vi "Send TDF File List Response.vi"(8 "error in (no error)":errorcluster caption="에러 입력(에러 없음)", 9 "TDF File List":string[](array[string]), 10 "id":string, 11 "Instrument Manager 입력":refnum<class "Instrument Manager.lvclass">) -> (0 "error out":errorcluster caption="에러 출력", 3 "Instrument Manager 출력":refnum<class "Instrument Manager.lvclass">)   [LabVIEW 2023, in "Instrument Manager.lvclass"]
uses:
  Instrument Manager.lvclass
  TDF File List Response.ctl
  Instrument Manager.lvclass/Instrument Manager.ctl
  Error Response.ctl
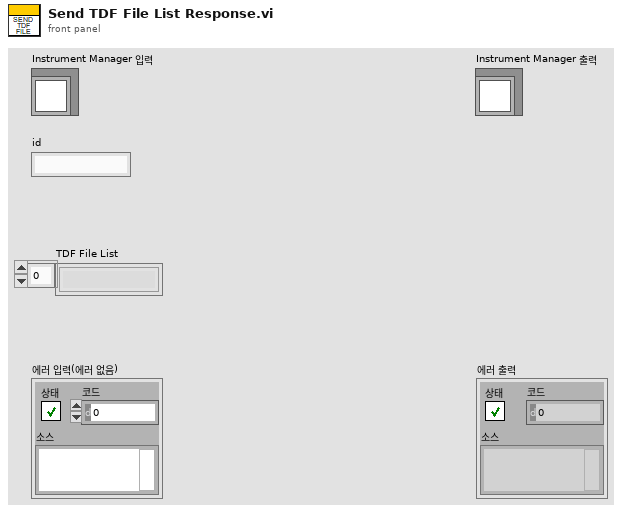
[diagram p1: front panel]
types:
  T1 = typedef "Instrument Manager.lvclass/TDF File List Response.ctl" = cluster{"type":string, "id":string, "status":string, "Result":cluster{"TDF File List":string[]}}
  T2 = cluster{"Reader Q":refnum<queue>, "Writer Q":refnum<queue>}
  T3 = typedef "Instrument Manager.lvclass/Error Response.ctl" = cluster{"type":string, "id":string, "status":string, "error out":errorcluster}
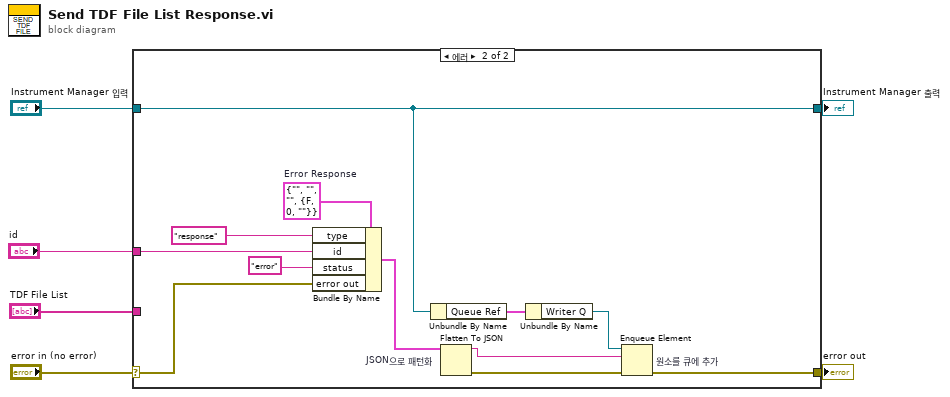
[diagram p0: block diagram]
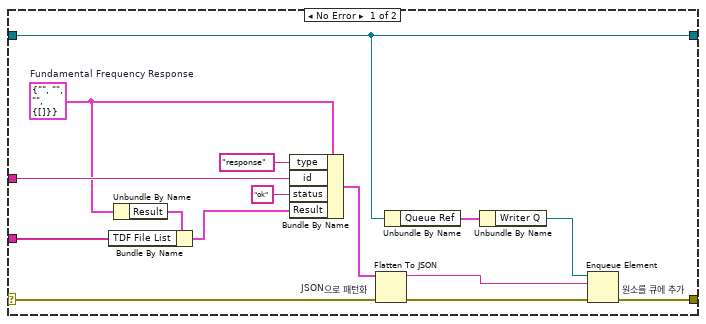
[diagram p2: hidden frame]
diagram:
  n1 = case shown="에러" "error in (no error)" {
    selector: "error in (no error)" -> [w13 w24]
    tunnel: [w14 w25] -> w5
    tunnel: [w7 w22] -> w3
    tunnel: "Instrument Manager 입력" -> [w7 w22]
    tunnel: "id" -> [w15 w23]
    tunnel: "TDF File List" -> [w8 _]
    frame No Error {
      w12 = T1 {"type"="", "id"="", "status"="", "Result"={"TDF File List"=[]}}  # Fundamental Frequency Response
      n2 = Unbundle By Name(w12) -> ("Result"=w11:cluster{"TDF File List":string[]})
      n3 = Bundle By Name(cluster=w11, "TDF File List"=w8) -> (w9:cluster{"TDF File List":string[]})
      n4 = Bundle By Name(cluster=w12, "type"="response", "id"=w15, "status"="ok", "Result"=w9) -> (w16:T1)
      n5 = Flatten To JSON "JSON으로 패턴화"(anything=w16, error in (no error)=w13) -> (JSON string=w17:string, 11:w10:errorcluster)  [unwired: 1 in]
      n6 = Unbundle By Name(w7) -> ("Queue Ref"=w19:T2)
      n7 = Unbundle By Name(w19) -> ("Writer Q"=w18:refnum<queue>)
      n8 = Enqueue Element "원소를 큐에 추가"(queue=w18, element=w17, error in (no error)=w10) -> (error out=w14:errorcluster)  [unwired: 1 in, 2 out]
    }
    frame Error {
      w33 = T3 {"type"="", "id"="", "status"="", "error out"={"status"=FALSE, "code"=0, "source"=""}}  # Error Response
      n9 = Bundle By Name(cluster=w33, "type"="response", "id"=w23, "status"="error", "error out"=w24) -> (w29:T3)
      n10 = Unbundle By Name(w22) -> ("Queue Ref"=w27:T2)
      n11 = Flatten To JSON "JSON으로 패턴화"(anything=w29) -> (JSON string=w32:string, 11:w28:errorcluster)  [unwired: 2 in]
      n12 = Unbundle By Name(w27) -> ("Writer Q"=w26:refnum<queue>)
      n13 = Enqueue Element "원소를 큐에 추가"(queue=w26, element=w32, error in (no error)=w28) -> (error out=w25:errorcluster)  [unwired: 1 in, 2 out]
    }
  }
  "error out" <- w5
  "Instrument Manager 출력" <- w3
